vi "Register For Events.vi"(8 "error in (no error)":errorcluster, 11 "ToastService in":refnum<class "ToastService.lvclass">) -> (0 "error out":errorcluster, 3 "ToastService out":refnum<class "ToastService.lvclass">)   [LabVIEW 2026, in "ToastNotification.lvlib" / "ToastService.lvclass"]
doc: "Registers the notification manager’s OnActivated callback and stores its registration reference in ToastService. Call after Initialize and before Show. If a callback is already registered, returns error 550016 and preserves the existing registration so Close can unregister it. On incoming error, skips registration and passes the service and error through unchanged."
uses:
  ToastService.lvclass
  ToastService.lvclass/ToastService.ctl
  Read ActivationHandler.vi
  Write event callback refnum.vi
  CallBack VI - OnActivated.vi
  Read reference.vi
  Write reference.vi
  ActivationHandler/ActivationHandler.lvclass
  <vilib>/ErrorRing/Error Ring.xnode
  <vilib>/Utility/error.llb/Error Cluster From Error Code.vi
  C:/Users/loicw/Documents/LabVIEW/ToastNotifications/Sources/bins/Microsoft.Toolkit.Uwp.Notifications.dll
  bins/Microsoft.Toolkit.Uwp.Notifications.dll
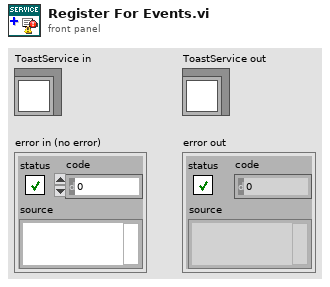
[diagram p1: front panel]
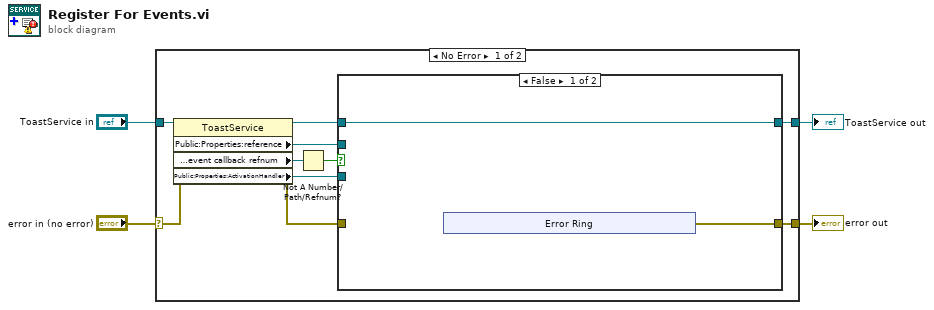
[diagram p0: block diagram]
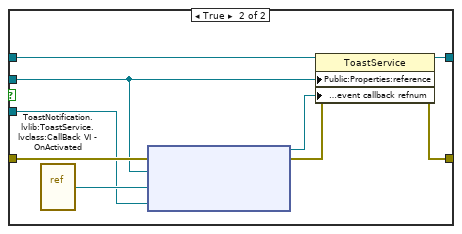
[diagram p2: hidden frame]
diagram:
  n1 = case shown="No Error" "error in (no error)" {
    selector: "error in (no error)" -> [w12 w32]
    tunnel: [w8 w32] -> w3
    tunnel: [w10 w31] -> w1
    tunnel: "ToastService in" -> [w14 w31]
    frame No Error {
      n2 = property class="ToastService"(reference=w14, error in=w12) -> (reference out=w13:refnum<class "ToastService.lvclass">, error out=w11:errorcluster, "Public:Properties:reference"=w9:refnum<k24>, "Private:Properties:event callback refnum"=w5:refnum<k27>, "Public:Properties:ActivationHandler"=w7:refnum<class "ActivationHandler.lvclass">)
      n3 = Not A Number/Path/Refnum?(number/path/refnum=w5) -> (NaN/Path/Refnum?=w6:bool)
      n4 = case shown="False" w6 {
        tunnel: w13 -> [w16 w30]
        tunnel: w11 -> [_ w29]
        tunnel: [w16 w28] -> w10
        tunnel: w9 -> [_ w27]
        tunnel: [w15 w25] -> w8
        tunnel: w7 -> [_ w22]
        frame False {
          n5 = xnode "Error Ring"() -> ("error out"=w15:errorcluster)
        }
        frame True {
          n6 = vi-ref "ToastNotification.lvlib:ToastService.lvclass:CallBack VI - OnActivated.vi"() -> ("vi reference"=w23:refnum<vi>)
          n7 = node(w29, w27, w23, w22) -> (w24:refnum<k27>, w26:errorcluster)  [unwired: 1 in]
          n8 = property class="ToastService"(reference=w30, error in=w26, "Public:Properties:reference"=w27, "Private:Properties:event callback refnum"=w24) -> (reference out=w28:refnum<class "ToastService.lvclass">, error out=w25:errorcluster)
        }
      }
    }
    frame Error {
    }
  }
  "error out" <- w3
  "ToastService out" <- w1
